vi "Limit AO Amplitude.vi"(8 "error in (no error)":errorcluster, 11 "Instrument.DAQ":refnum<class "Instrument.DAQ.lvclass">) -> (0 "error out":errorcluster, 3 "Instrument.DAQ out":refnum<class "Instrument.DAQ.lvclass">)   [LabVIEW 2019, in "Instrument.Lockin.lvlib" / "Instrument.DAQ.lvclass"]
uses:
  Instrument.DAQ.lvclass
  Instrument.DAQ.lvclass/Instrument.DAQ.ctl
  74a9887d-d73a-48f6-ba86-af19fb548ebb.vi
panel:
  # "2"
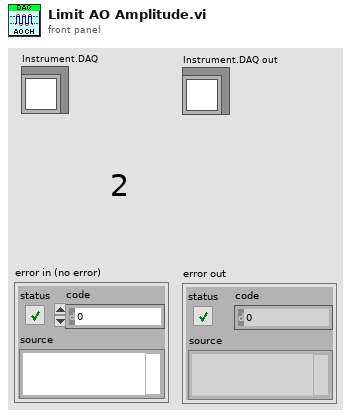
[diagram p1: front panel]
types:
  T1 = typedef "Instrument.Lockin.lvlib/Instrument.DAQ.lvclass/AO.Channel--Cluster--Array.ctl" = T2[]
  T2 = typedef "Instrument.Lockin.lvlib/Instrument.DAQ.lvclass/AO.Channel--Cluster.ctl" = cluster{"Enable?":bool, "Channel":i32, "Amplitude":dbl, "Offset":dbl, "Frequency":dbl, "Phase":dbl, "Function":T3, "Sweeping?":bool, "Limit AC":bool, "Limit DC?":bool}
  T3 = typedef "Instrument.Lockin.lvlib/Instrument.DAQ.lvclass/AO.Channel.Function--Enum.ctl" = enum16{"Sine", "Triangle", "Square"}
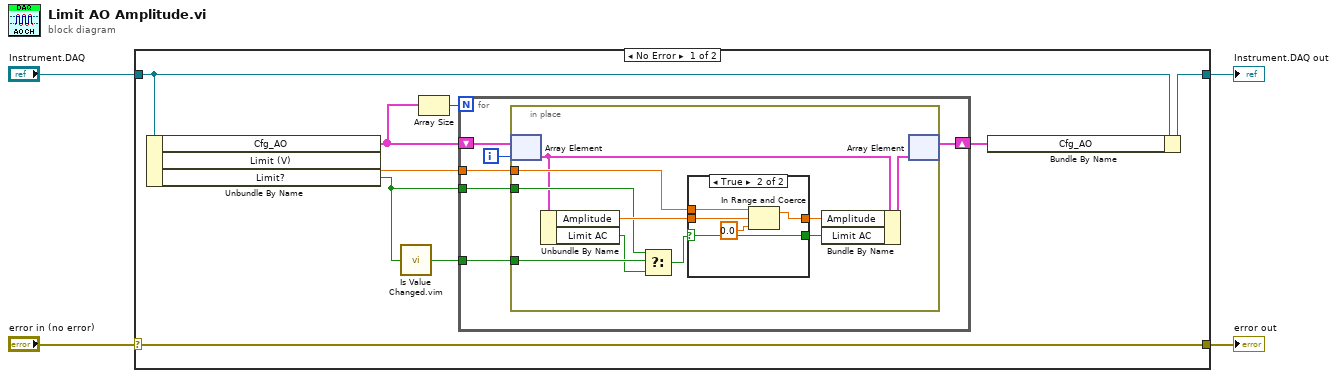
[diagram p0: block diagram]
diagram:
  n1 = case shown="No Error" "error in (no error)" {
    selector: "error in (no error)" -> [w10 w38]
    tunnel: [w13 w37] -> w4
    tunnel: "Instrument.DAQ" -> [w12 w37]
    tunnel: [w10 w38] -> w2
    frame No Error {
      n2 = Unbundle By Name(w12) -> ("Cfg_AO"=w5:T1, "Limit (V)"=w9:dbl, "Limit?"=w8:bool)
      n3 = call "Is Value Changed.vim"("value"=w8) -> ("changed or first call?"=w7:bool)
      n4 = Array Size(array=w5) -> (size(s)=w6:i32)
      n5 = for {
        N: w6 -> [_]
        tunnel: w9 -> [w19]
        tunnel: w7 -> [w18]
        tunnel: w8 -> [w17]
        shift-right: [w15] -> w11
        shift-left: w5 -> [w16]
        i -> [w14]
        n6 = in-place {
          in-place-border: w19 -> [w26]
          in-place-border: w18 -> [w25]
          in-place-border: w17 -> [w24]
          n7 = in-place-array #1(w16, w14) -> (w21:T2)
          n8 = Unbundle By Name(w21) -> ("Amplitude"=w29:dbl, "Limit AC"=w23:bool)
          n9 = Select(t=w24, s=w25, f=w23) -> (s? t:f=w22:bool)
          n10 = case shown="True" w22 {
            selector: w22 -> [w30 w33]
            tunnel: w29 -> [w31 w35]
            tunnel: w26 -> [_ w32]
            tunnel: [w31 w34] -> w28
            tunnel: [w30 w33] -> w27
            frame False {
            }
            frame True {
              n11 = In Range and Coerce(upper limit=w32, x=w35, lower limit=0.0) -> (coerced(x)=w34:dbl)  [unwired: 1 out]
            }
          }
          n12 = Bundle By Name(cluster=w21, "Amplitude"=w28, "Limit AC"=w27) -> (w20:T2)
          n13 = in-place-array #1(w20) -> (w15:T1)  [unwired: 1 out]
        }
      }
      n14 = Bundle By Name(cluster=w12, "Cfg_AO"=w11) -> (w13:refnum<class "Instrument.DAQ.lvclass">)
    }
    frame Error {
    }
  }
  "Instrument.DAQ out" <- w4
  "error out" <- w2
